vi "clear status flag.vi"(8 "error in (no error)":errorcluster, 10 "flag name to clear":string, 11 "flag to clear":u32 format="%x") -> (0 "error out":errorcluster, 3 "cleared":bool)   [LabVIEW 2024, in "atsj peakcan basic.lvlib"]
uses:
  atsj peakcan basic.lvlib
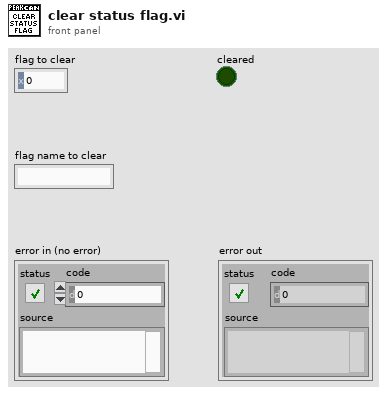
[diagram p1: front panel]
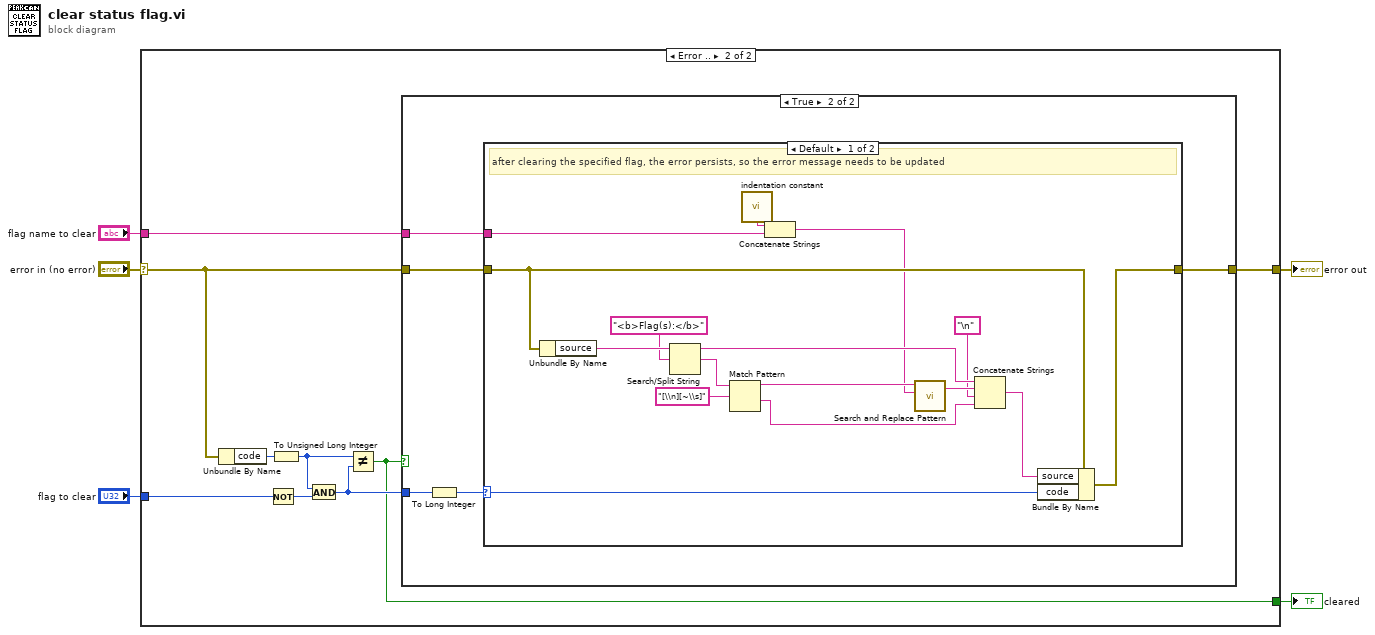
[diagram p0: block diagram]
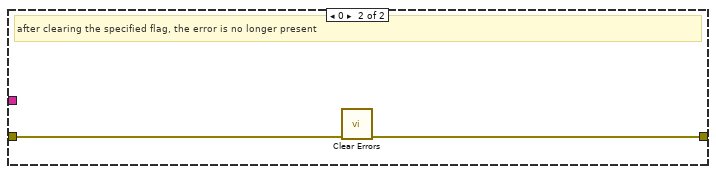
[diagram p4: hidden frame]
diagram:
  n1 = case shown="Error .." "error in (no error)" {
    selector: "error in (no error)" -> [w6 w9]
    tunnel: "flag to clear" -> [_ w14]
    tunnel: "flag name to clear" -> [_ w10]
    tunnel: [w6 w8] -> w2
    tunnel: [_ w7] -> w1
    frame No Error {
    }
    frame Error {
      n2 = Unbundle By Name(w9) -> ("code"=w12:i32)
      n3 = Not(x=w14) -> (.not. x?=w15:u32)
      n4 = To Unsigned Long Integer(number=w12) -> (unsigned 32bit integer=w13:u32)
      n5 = And(x=w13, y=w15) -> (x .and. y?=w11:u32)
      n6 = Not Equal?(x=w13, y=w11) -> (x != y?=w7:bool)
      n7 = case shown="True" w7 {
        tunnel: w9 -> [w16 w19]
        tunnel: w11 -> [_ w21]
        tunnel: [w16 w18] -> w8
        tunnel: w10 -> [_ w17]
        frame False {
        }
        frame True {
          n8 = To Long Integer(number=w21) -> (32bit integer=w20:i32)
          n9 = case shown="Default" w20 {
            selector: w20 -> [w28 _]
            tunnel: w19 -> [w30 w39]
            tunnel: [w29 w38] -> w18
            tunnel: w17 -> [w32 _]
            frame Default {
              # "after clearing the specified flag, the error persists, so the error message needs to be updated"
              n10 = Unbundle By Name(w30) -> ("source"=w37:string)
              n11 = Search/Split String(string=w37, search string/char (-)="<b>Flag(s):</b>") -> (substring before match=w25:string, match + rest of string=w35:string)  [unwired: 1 in, 1 out]
              n12 = Match Pattern(string=w35, regular expression="[\\n][~\\s]") -> (before substring=w36:string, after substring=w26:string)  [unwired: 1 in, 2 out]
              n13 = call "indentation constant.vi"() -> ("indentation"=w31:string)
              n14 = Concatenate Strings(w31, w32) -> (w22:string)
              n15 = call <vilib>:"Search and Replace Pattern.vi"("string"=w36, "regular expression (\"\")"=w22) -> ("result string"=w27:string)  [unwired: 3 in, 1 out]
              n16 = Concatenate Strings(w25, w27, "\n", w26) -> (w24:string)
              n17 = Bundle By Name(cluster=w30, "source"=w24, "code"=w28) -> (w29:errorcluster)
            }
            frame 0 {
              # "after clearing the specified flag, the error is no longer present"
              n18 = call <vilib>:"Clear Errors.vi"("error in (no error)"=w39) -> ("error out"=w38:errorcluster)  [unwired: 5 in, 1 out]
            }
          }
        }
      }
    }
  }
  "error out" <- w2
  "cleared" <- w1
